vi "Set ThermalChamberController SubscribeChamberStatusUpdated Response.vi"(7 "Streaming? (F)":bool, 8 "error in (no error)":errorcluster, 10 "Message Data":T1, 11 "gRPCid in":T3) -> (0 "error out":errorcluster)   [LabVIEW 2020, in "thermal-chamber-controller_server.lvlib" / "ThermalChamberController.lvclass"]
uses:
  ThermalChamberController.lvclass
  <vilib>/gRPC/LabVIEW gRPC Library/Shared/grpcId.ctl
  ThermalChamberController.lvclass/ThermalChamberController.ctl
  thermal-chamber-controller_server.lvlib
  <vilib>/gRPC/LabVIEW gRPC Library/grpc-lvsupport-release.lvlib
  RPC Messages/lv_python_grpc_webui_demo_v1_HeaterState.ctl
  RPC Messages/lv_python_grpc_webui_demo_v1_ChamberStatus.ctl
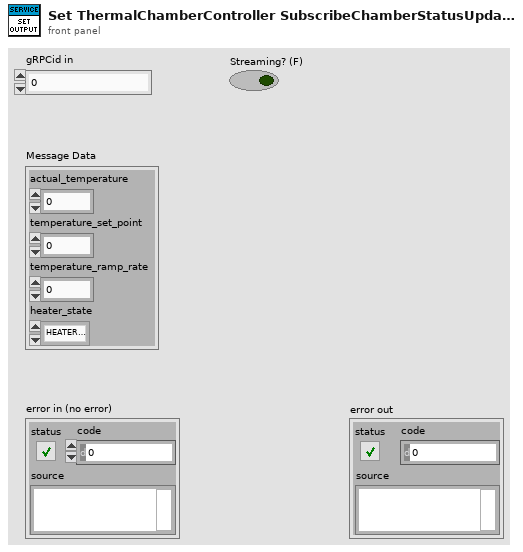
[diagram p1: front panel]
types:
  T1 = typedef "thermal-chamber-controller_server.lvlib/lv_python_grpc_webui_demo_v1_ChamberStatus.ctl" = cluster{"actual_temperature":dbl, "temperature_set_point":dbl, "temperature_ramp_rate":dbl, "heater_state":T2}
  T2 = typedef "thermal-chamber-controller_server.lvlib/lv_python_grpc_webui_demo_v1_HeaterState.ctl" = enum32{"HEATER_ENABLED", "HEATER_DISABLED"}
  T3 = typedef "grpc-lvsupport-release.lvlib/grpcId.ctl" = u64
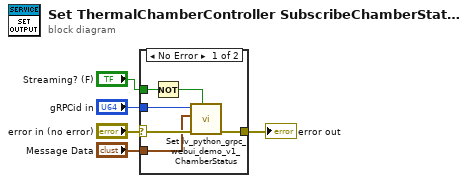
[diagram p0: block diagram]
diagram:
  n1 = case shown="No Error" "error in (no error)" {
    selector: "error in (no error)" -> [w11 w12]
    tunnel: [w9 w12] -> w4
    tunnel: "gRPCid in" -> [w10 _]
    tunnel: "Message Data" -> [w8 _]
    tunnel: "Streaming? (F)" -> [w7 _]
    frame No Error {
      n2 = Not(x=w7) -> (.not. x?=w6:bool)
      n3 = call "Set lv_python_grpc_webui_demo_v1_ChamberStatus.vi"("Complete Call (T)"=w6, "error in (no error)"=w11, "package_templatemessage"=w8, "gRPCid"=w10) -> ("error out"=w9:errorcluster)  [unwired: 7 in]
    }
    frame Error {
    }
  }
  "error out" <- w4
